vi "test streamed tool error.vi"(8 "error in (no error)":errorcluster) -> (0 "error out":errorcluster, 3 "body":string)   [LabVIEW 2020, in "MCP Server tests.lvlib"]
doc: "A tools/call that fails while it is streamed (params._meta.progressToken and Accept: text/event-stream) is answered as text/event-stream whose last data event is the JSON-RPC answer with the request id, and the server answers the next request. Checked for an unknown tool (error -32602), and for fake_tool_add with an argument of the wrong type (result with isError true), each in the legacy era and the modern era (MCP 2026-07-28: params._meta with io.modelcontextprotocol/protocolVersion 2026-07-28 and clientCapabilities {}, headers MCP-Protocol-Version: 2026-07-28, Mcp-Method: tools/call, Mcp-Name: <tool name>). Before the fix such a call opened LabVIEW's error dialog in the background, the stream stayed empty and every later request timed out."
uses:
  MCP Server tests.lvlib
  <vilib>/addons/_JKI Toolkits/Caraya/classes/Test/Test.lvclass
  <vilib>/addons/_JKI Toolkits/Caraya/classes/Assert/Assert.lvclass
panel:
  out "lookup error":errorcluster
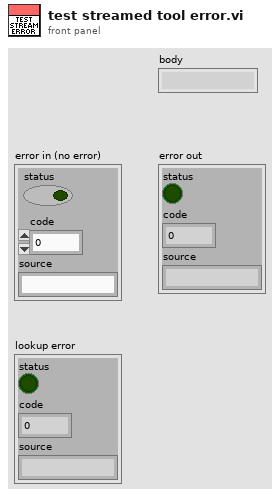
[diagram p1: front panel]
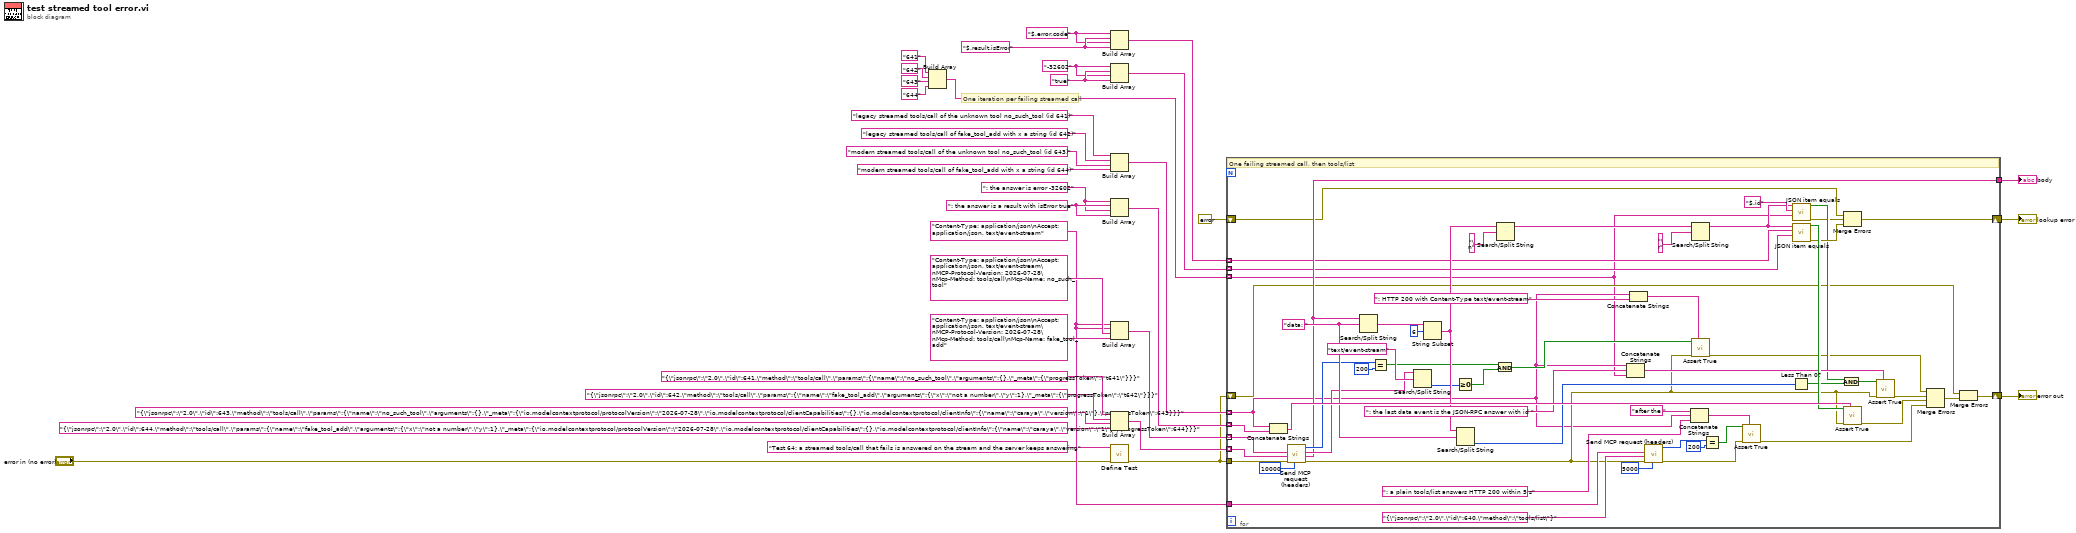
[diagram p0: block diagram]
diagram:
  w33 = ": the answer is a result with isError true" ("check isError")
  w32 = ": the answer is error -32602" ("check code")
  w25 = "true" ("expected isError")
  w24 = "-32602" ("expected code")
  w22 = "$.result.isError" ("isError path")
  w21 = "$.error.code" ("error code path")
  w12 = "Content-Type: application/json\nAccept: application/json, text/event-stream" ("legacy headers")
  # "One iteration per failing streamed call"
  n1 = Build Array("641" ("id 641"), "642" ("id 642"), "643" ("id 643"), "644" ("id 644")) -> (w20:string[])
  n2 = Build Array(w21, w22, w21, w22) -> (w23:string[])
  n3 = Build Array(w24, w25, w24, w25) -> (w26:string[])
  n4 = Build Array("legacy streamed tools/call of the unknown tool no_such_tool (id 641)" ("label 641"), "legacy streamed tools/call of fake_tool_add with x a string (id 642)" ("label 642"), "modern streamed tools/call of the unknown tool no_such_tool (id 643)" ("label 643"), "modern streamed tools/call of fake_tool_add with x a string (id 644)" ("label 644")) -> (w31:string[])
  n5 = Build Array(w32, w33, w32, w33) -> (w34:string[])
  n6 = Build Array(w12, w12, "Content-Type: application/json\nAccept: application/json, text/event-stream\nMCP-Protocol-Version: 2026-07-28\nMcp-Method: tools/call\nMcp-Name: no_such_tool" ("modern headers unknown tool"), "Content-Type: application/json\nAccept: application/json, text/event-stream\nMCP-Protocol-Version: 2026-07-28\nMcp-Method: tools/call\nMcp-Name: fake_tool_add" ("modern headers add")) -> (w15:string[])
  n7 = Build Array("{\"jsonrpc\":\"2.0\",\"id\":641,\"method\":\"tools/call\",\"params\":{\"name\":\"no_such_tool\",\"arguments\":{},\"_meta\":{\"progressToken\":\"t641\"}}}" ("request 641"), "{\"jsonrpc\":\"2.0\",\"id\":642,\"method\":\"tools/call\",\"params\":{\"name\":\"fake_tool_add\",\"arguments\":{\"x\":\"not a number\",\"y\":1},\"_meta\":{\"progressToken\":\"t642\"}}}" ("request 642"), "{\"jsonrpc\":\"2.0\",\"id\":643,\"method\":\"tools/call\",\"params\":{\"name\":\"no_such_tool\",\"arguments\":{},\"_meta\":{\"io.modelcontextprotocol/protocolVersion\":\"2026-07-28\",\"io.modelcontextprotocol/clientCapabilities\":{},\"io.modelcontextprotocol/clientInfo\":{\"name\":\"caraya\",\"version\":\"1\"},\"progressToken\":643}}}" ("request 643"), "{\"jsonrpc\":\"2.0\",\"id\":644,\"method\":\"tools/call\",\"params\":{\"name\":\"fake_tool_add\",\"arguments\":{\"x\":\"not a number\",\"y\":1},\"_meta\":{\"io.modelcontextprotocol/protocolVersion\":\"2026-07-28\",\"io.modelcontextprotocol/clientCapabilities\":{},\"io.modelcontextprotocol/clientInfo\":{\"name\":\"caraya\",\"version\":\"1\"},\"progressToken\":644}}}" ("request 644")) -> (w11:string[])
  n8 = call <vilib>:"Define Test.vi"("error in (no error)"="error in (no error)", "Label (VI Title)"="Test 64: a streamed tools/call that fails is answered on the stream and the server keeps answering") -> ("error out"=w6:errorcluster)  [unwired: 8 in, 1 out]
  n9 = for {
    shift-right: [w48] -> w3
    shift-left: errorcluster {"status"=FALSE, "code"=0, "source"=""} ("no lookup error") -> [w47]
    tunnel: w12 -> [w88]
    tunnel: w11 -> [w36] mode=indexing
    tunnel: w15 -> [w37] mode=indexing
    tunnel: w20 -> [w38] mode=indexing
    tunnel: w23 -> [w39] mode=indexing
    tunnel: w26 -> [w40] mode=indexing
    tunnel: w31 -> [w41] mode=indexing
    tunnel: w34 -> [w42] mode=indexing
    tunnel: w6 -> [w43]
    shift-right: [w44] -> w4
    shift-left: w6 -> [w45]
    tunnel: [w51] -> w2
    w63 = "data: " ("data marker")
    # "One failing streamed call, then tools/list"
    n10 = Concatenate Strings(w41, w42) -> (w82:string)
    n11 = call "Send MCP request (headers).vi"("timeout (10000)"=10000 ("timeout"), "error in (no error)"=w43, "request"=w36, "request headers"=w37) -> ("error out"=w50:errorcluster, "response"=w51:string, "headers"=w52:string, "status code"=w53:i32)  [unwired: 4 in]
    n12 = Search/Split String(string=w51, search string/char (-)=w63) -> (match + rest of string=w64:string)  [unwired: 1 in, 2 out]
    n13 = Equal?(x=w53, y=200 ("expected 200")) -> (x = y?=w55:bool)
    n14 = Search/Split String(string=w52, search string/char (-)="text/event-stream" ("pattern")) -> (offset of match=w57:i32)  [unwired: 1 in, 2 out]
    n15 = String Subset(string=w64, offset (0)=6 ("after data:")) -> (substring=w66:string)  [unwired: 1 in]
    n16 = Greater Or Equal To 0?(x=w57) -> (x >= 0?=w58:bool)
    n17 = Search/Split String(string=w66, search string/char (-)=w63) -> (offset of match=w71:i32)  [unwired: 1 in, 2 out]
    n18 = And(x=w55, y=w58) -> (x .and. y?=w59:bool)
    n19 = Search/Split String(string=w66, search string/char (-)="\n" ("line feed")) -> (substring before match=w68:string)  [unwired: 1 in, 2 out]
    n20 = Concatenate Strings(w41, ": the last data event is the JSON-RPC answer with id " ("text 2"), w38) -> (w77:string)
    n21 = Concatenate Strings(w41, ": HTTP 200 with Content-Type text/event-stream" ("text 1")) -> (w61:string)
    n22 = call "Send MCP request (headers).vi"("timeout (10000)"=5000 ("5 s"), "error in (no error)"=w50, "request"="{\"jsonrpc\":\"2.0\",\"id\":640,\"method\":\"tools/list\"}" ("tools/list"), "request headers"=w88) -> ("error out"=w86:errorcluster, "status code"=w87:i32)  [unwired: 4 in, 2 out]
    n23 = Concatenate Strings("after the " ("after"), w41, ": a plain tools/list answers HTTP 200 within 5 s" ("text 4")) -> (w93:string)
    n24 = Search/Split String(string=w68, search string/char (-)="\r" ("carriage return")) -> (substring before match=w70:string)  [unwired: 1 in, 2 out]
    n25 = call <vilib>:"Assert True.vi"("Label"=w61, "error in (no error)"=w50, "True?"=w59) -> ("error out"=w62:errorcluster)  [unwired: 7 in, 1 out]
    n26 = Equal?(x=w87, y=200 ("expected 200")) -> (x = y?=w90:bool)
    n27 = call <vilib>:"Assert True.vi"("Label"=w93, "error in (no error)"=w86, "True?"=w90) -> ("error out"=w94:errorcluster)  [unwired: 7 in, 1 out]
    n28 = Less Than 0?(x=w71) -> (x < 0?=w72:bool)
    n29 = call "JSON item equals.vi"("expected"=w38, "path"="$.id" ("id path"), "JSON"=w70) -> ("error out"=w74:errorcluster, "equal?"=w75:bool)  [unwired: 6 in, 1 out]
    n30 = call "JSON item equals.vi"("expected"=w40, "path"=w39, "JSON"=w70) -> ("error out"=w80:errorcluster, "equal?"=w81:bool)  [unwired: 6 in, 1 out]
    n31 = And(x=w75, y=w72) -> (x .and. y?=w79:bool)
    n32 = Merge Errors(w47, w74, w80) -> (w48:errorcluster)
    n33 = call <vilib>:"Assert True.vi"("Label"=w82, "error in (no error)"=w50, "True?"=w81) -> ("error out"=w83:errorcluster)  [unwired: 7 in, 1 out]
    n34 = call <vilib>:"Assert True.vi"("Label"=w77, "error in (no error)"=w50, "True?"=w79) -> ("error out"=w78:errorcluster)  [unwired: 7 in, 1 out]
    n35 = Merge Errors(w62, w78, w83, w94) -> (w46:errorcluster)
    n36 = Merge Errors(w45, w46) -> (w44:errorcluster)
  }
  "body" <- w2
  "lookup error" <- w3
  "error out" <- w4
